vi "AverageFilter_Example.vi"() -> ()   [LabVIEW 2019]
uses:
  <vilib>/Rock Robotics/WPI/ThirdParty/JAS_Junk/TrajLib/Trajectory_Library.lvlib
  <vilib>/Rock Robotics/WPI/ThirdParty/JAS_Junk/TrajLib/LinearFilter_MovingAvg_Execute.vi
panel:
  in  "Auto / Manual\nProcess Variable\nGeneration":bool=TRUE
  in  "Enable\nNoise":bool=TRUE
  in  "Filter Enable":bool=TRUE
  in  "Use White Noise":bool=TRUE
  in  "Tab Control 2":enum32{"Avg 3", "Avg 7"}(tab)
  out "Avg3":cluster{dbl, dbl, "Value_Output":dbl}(graph)
  out "Avg3 Out Dial":dbl(knob)=-2.895988890827539e-05 scale=-20.0..20.0
  out "Avg3 Out":dbl format="%11.3f"
  out "Avg7":cluster{dbl, dbl, "Value_Output":dbl}(graph)
  out "Avg7 Out":dbl format="%11.3f"
  out "Avg7 Out Dial":dbl(knob)=-2.895988890827539e-05 scale=-20.0..20.0
  out "Loop Adjust":dbl format="%11.3f"
  in  "Manual\nInput":dbl(slide) min=-12.0 max=12.0 scale=-12.0..12.0
  out "Raw Noise":dbl(knob)=-2.895988890827539e-05 scale=-20.0..20.0
  out "Raw Noise":dbl format="%11.3f"
  out "Actual Input":dbl(knob)=-2.895988890827539e-05 scale=-20.0..20.0
  out "Actual Input":dbl format="%11.3f"
  out "Input":cluster{"Manual\nInput":dbl, dbl, "f":dbl}(graph)
  out "Meas Dial":dbl(knob)=-2.895988890827539e-05 scale=-20.0..20.0
  out "Measured Value":dbl format="%11.3f"
  # "Average Filter Example"
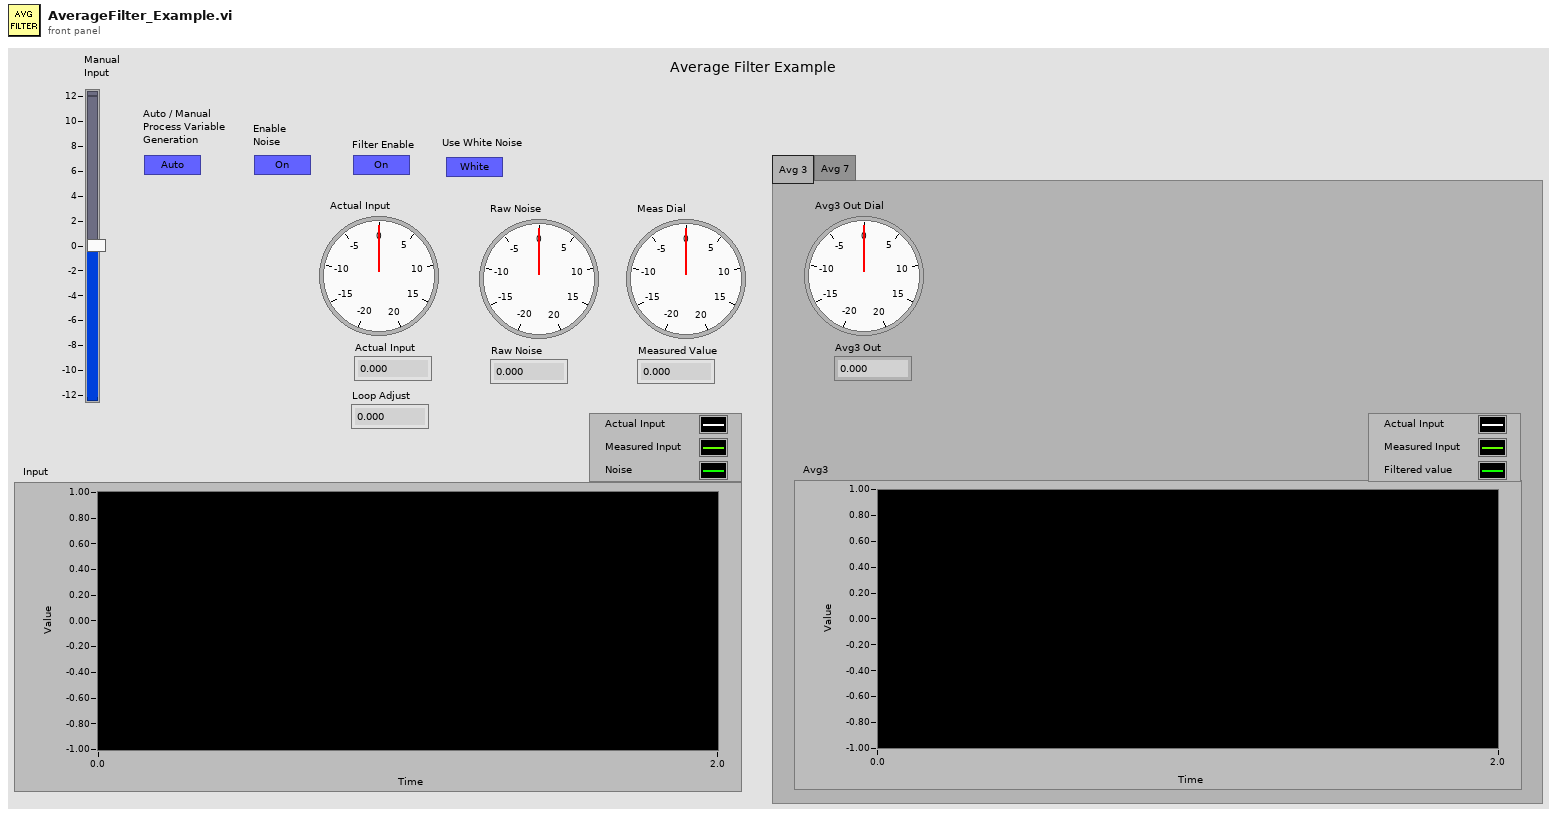
[diagram p1: front panel]
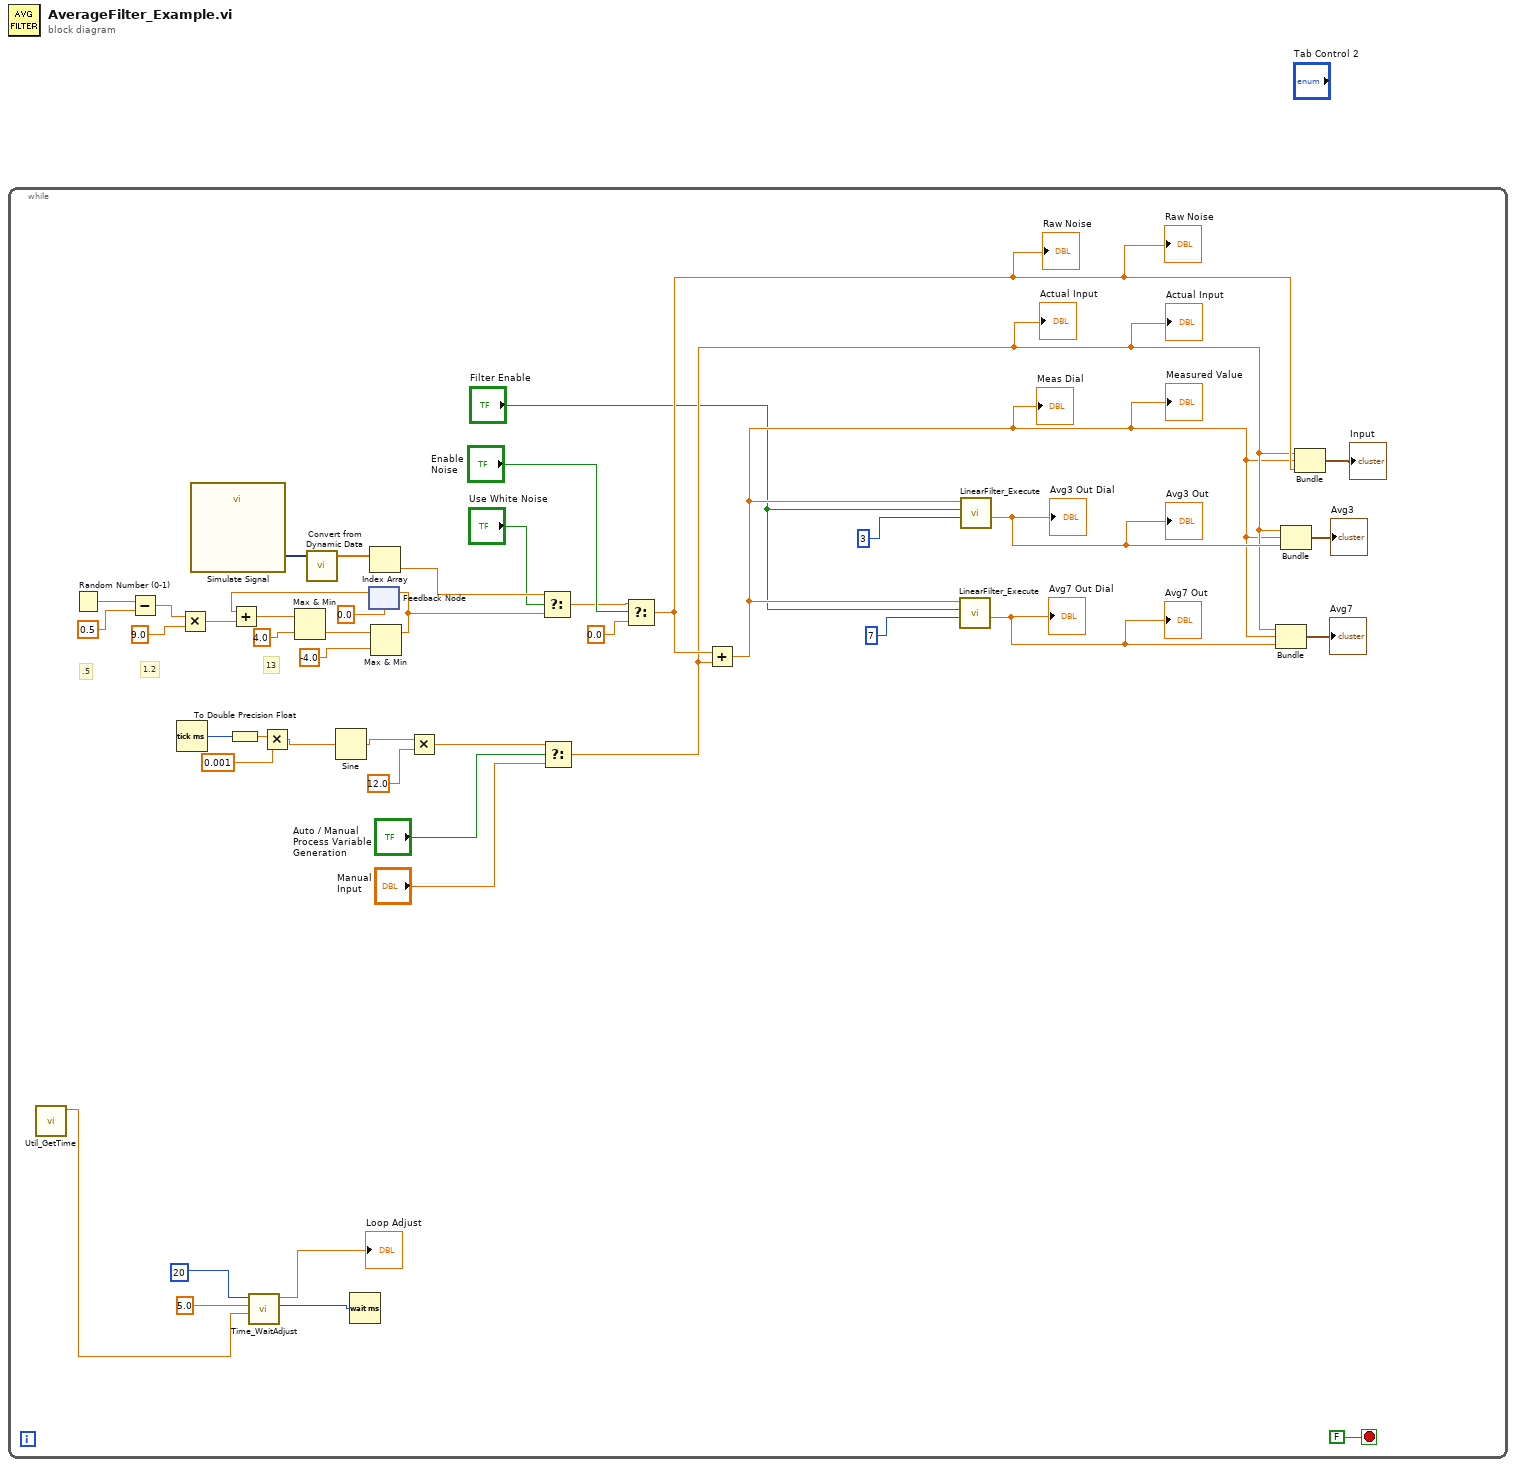
[diagram p0: block diagram]
diagram:
  n1 = while {
    stop <- FALSE stop-if-true
    # "13"
    # "1.2"
    # ".5"
    n2 = call <vilib>:"Util_GetTime.vi"() -> ("FPGA_Time_Seconds"=w2:dbl)  [unwired: 9 in, 2 out]
    n3 = Random Number (0-1)() -> (number: 0 to 1=w40:dbl)
    n4 = Subtract(x=w40, y=0.5) -> (x-y=w36:dbl)
    n5 = Tick Count (ms)() -> (millisecond timer value=w31:u32)
    n6 = Multiply(x=w36, y=9.0) -> (x*y=w35:dbl)
    n7 = call "Simulate Signal"() -> ("DC with Uniform Noise"=w19:dynamicdata)  [unwired: 14 in, 1 out]
    n8 = To Double Precision Float(number=w31) -> (double precision float=w32:dbl)
    n9 = call <vilib>:"Time_WaitAdjust.vi"("PassthroughTime_SEC"=w2, "MaxAdjustment_MS"=5.0 ("MaxDeviation_MS"), "DesiredLoopTime_MS"=u32 20 ("milliseconds to wait")) -> ("AdjustedWaitTime_MS"=w4:u32, "Offset_MS"=→"Loop Adjust":dbl)  [unwired: 7 in]
    n10 = Multiply(x=w32, y=0.001) -> (x*y=w29:dbl)
    n11 = call "Convert from Dynamic Data"("Dynamic Data Type"=w19) -> ("Array"=w18:dbl[])  [unwired: 3 in]
    n12 = Sine(x=w29) -> (sin(x)=w28:dbl)
    n13 = Wait (ms)(milliseconds to wait=w4) -> ()  [unwired: 1 out]
    n14 = feedback #1(0.0) -> (w37:dbl)
    n15 = Add(x=w37, y=w35) -> (x+y=w39:dbl)
    n16 = Max & Min(x=w39, y=4.0) -> (min(x,y)=w38:dbl)  [unwired: 1 out]
    n17 = Index Array(array=w18) -> (element=w17:dbl)  [unwired: 1 in]
    n18 = Max & Min(x=w38, y=-4.0) -> (max(x,y)=w20:dbl)  [unwired: 1 out]
    n19 = feedback-in #1(w20) -> ()
    n20 = Multiply(x=w28, y=12.0) -> (x*y=w25:dbl)
    n21 = Select(t=w17, s="Use White Noise", f=w20) -> (s? t:f=w21:dbl)
    n22 = Select(t=w25, s="Auto / Manual\nProcess Variable\nGeneration", f="Manual\nInput") -> (s? t:f=w8:dbl)
    "Actual Input" <- w8
    "Actual Input" <- w8
    n23 = Select(t=w21, s="Enable\nNoise", f=0.0) -> (s? t:f=w15:dbl)
    "Raw Noise" <- w15
    "Raw Noise" <- w15
    n24 = Add(x=w15, y=w8) -> (x+y=w7:dbl)
    "Measured Value" <- w7
    "Meas Dial" <- w7
    n25 = call-poly <vilib>:"LinearFilter_Execute.vi"("Samples"=7, "Enable"="Filter Enable", "Input"=w7) -> ("Output"=w12:dbl)  [unwired: 8 in]
    "Avg7 Out" <- w12
    "Avg7 Out Dial" <- w12
    n26 = call-poly <vilib>:"LinearFilter_Execute.vi"("Samples"=3, "Enable"="Filter Enable", "Input"=w7) -> ("Output"=w13:dbl)  [unwired: 8 in]
    "Avg3 Out" <- w13
    "Avg3 Out Dial" <- w13
    n27 = Bundle("Manual\nInput"=w8, w7, "Output"=w12) -> (→"Avg7":cluster{"Manual\nInput":dbl, dbl, "Output":dbl})  [unwired: 1 in]
    n28 = Bundle("Manual\nInput"=w8, w7, "Output"=w13) -> (→"Avg3":cluster{"Manual\nInput":dbl, dbl, "Output":dbl})  [unwired: 1 in]
    n29 = Bundle("Manual\nInput"=w8, w7, "f"=w15) -> (→"Input":cluster{"Manual\nInput":dbl, dbl, "f":dbl})  [unwired: 1 in]
  }
